vi "RT_lab8.vi"() -> ()   [LabVIEW 2025]
uses:
  states.ctl
panel:
  out "Elements Remaining":u32
  out "Waveform Graph":i16[][](graph)
  out "error out":errorcluster
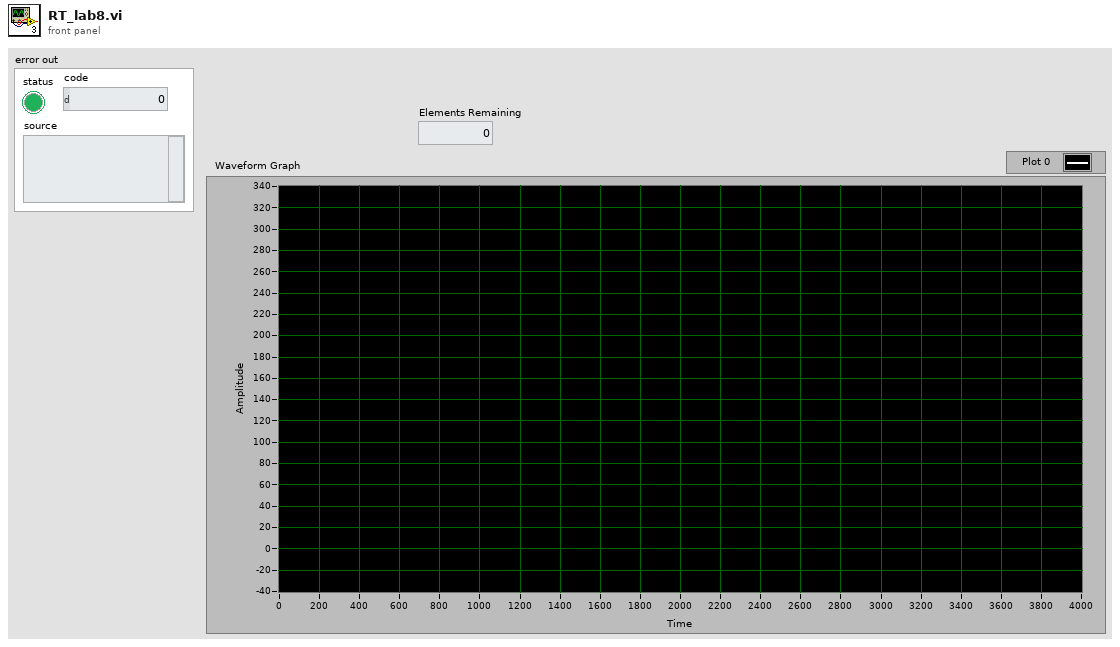
[diagram p1: front panel]
types:
  T1 = typedef "states.ctl" = enum16{"Run", "Connect"}
  T2 = typedef "RT_Cmd.ctl" = cluster{"command":T3, "parameters":T4}
  T3 = typedef "Command.ctl" = enum16{"threshold_config", "manual_trigger", "stop"}
  T4 = typedef "thresholds.ctl" = cluster{"Thr_X":i16, "Thr_Y":i16, "Thr_Z":i16}
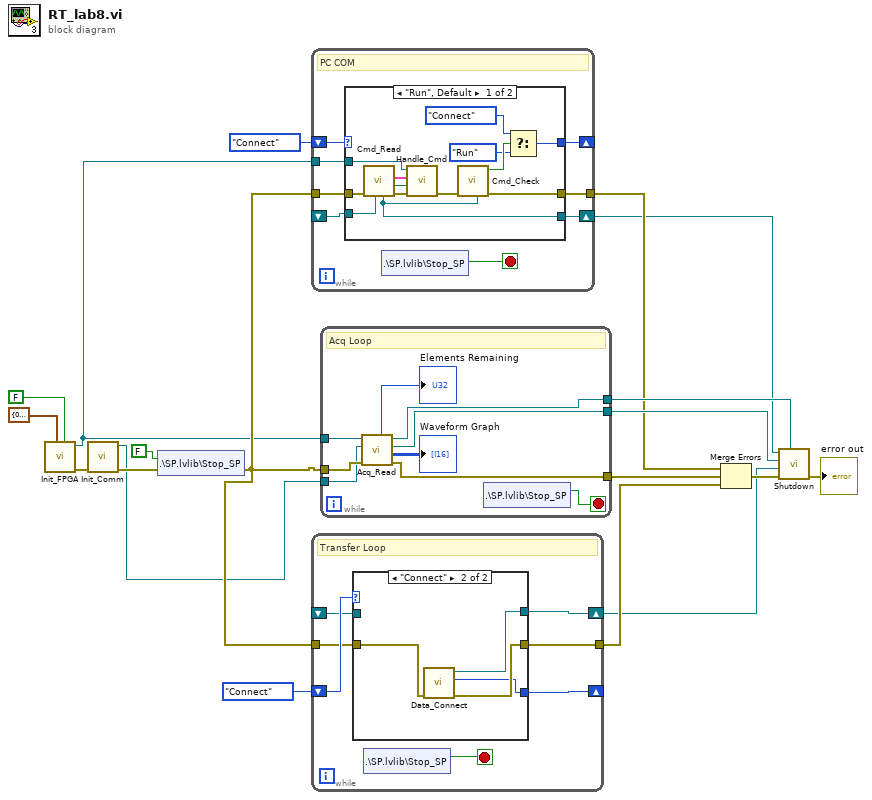
[diagram p0: block diagram]
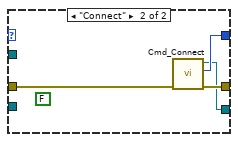
[diagram p2: hidden frame]
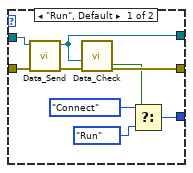
[diagram p3: hidden frame]
diagram:
  n1 = call "Init_FPGA.vi"("manual trigger"=FALSE, "Threshold"=cluster{"Thr_X":i16, "Thr_Y":i16, "Thr_Z":i16} {"Thr_X"=0, "Thr_Y"=0, "Thr_Z"=0}) -> ("error out"=w18:errorcluster, "FPGA VI Reference Out"=w8:refnum<k20>)  [unwired: 8 in]
  n2 = call "Init_Comm.vi"("error in"=w18) -> ("error out"=w14:errorcluster, "rt fifo ref out"=w11:refnum<k33>)  [unwired: 9 in]
  n3 = shared-variable ".\\SP.lvlib\\Stop_SP"(FALSE ("Stop_SP"), error in=w14) -> (error out=w12:errorcluster)
  n4 = while {
    tunnel: w12 -> [w26]
    tunnel: w8 -> [w25]
    shift-right: [w24] -> _
    shift-left: states."Connect" -> [w27]
    tunnel: [w23] -> w3
    shift-right: [w22] -> w1
    shift-left: _ -> [w21]
    stop <- w20 stop-if-true
    # "PC COM"
    n5 = case shown="\"Run\", Default" w27 {
      tunnel: w26 -> [w40 w44]
      tunnel: w25 -> [w38 _]
      tunnel: [w39 w43] -> w23
      tunnel: [w28 w42] -> w24
      tunnel: [w32 w41] -> w22
      tunnel: w21 -> [w33 _]
      frame "Run", Default {
        n6 = call "Cmd_Read.vi"("Refnum in"=w33, "error in (no error)"=w40) -> ("error out"=w35:errorcluster, "timed out?"=w36:bool, "data out"=w37:T2, "Refnum out"=w32:refnum<k21>)  [unwired: 6 in]
        n7 = call "Handle_Cmd.vi"("error in"=w35, "timed out?"=w36, "data IN"=w37, "FPGA VI Reference IN"=w38) -> ("error out"=w34:errorcluster)  [unwired: 6 in, 1 out]
        n8 = call "Cmd_Check.vi"("Refnum in"=w32, "error in (no error)"=w34) -> ("error out"=w39:errorcluster, "disconnected?"=w31:bool)  [unwired: 8 in]
        n9 = Select(t=states."Connect", s=w31, f=states."Run") -> (s? t:f=w28:T1)
      }
      frame "Connect" {
        (unwired) FALSE
        n10 = call "Cmd_Connect.vi"("error in (no error)"=w44) -> ("error out"=w43:errorcluster, "Enum"=w42:T1, "Refnum out"=w41:refnum<k21>)  [unwired: 8 in]
      }
    }
    n11 = shared-variable ".\\SP.lvlib\\Stop_SP"() -> (w20:bool)  [unwired: 1 in, 1 out]
  }
  n12 = while {
    tunnel: w12 -> [w48]
    shift-right: [w47] -> _
    shift-left: states."Connect" -> [w51]
    shift-right: [w50] -> w2
    shift-left: _ -> [w49]
    tunnel: [w46] -> w5
    stop <- w45 stop-if-true
    # "Transfer Loop"
    n13 = case shown="\"Connect\"" w51 {
      tunnel: [w56 w61] -> w50
      tunnel: w49 -> [w59 _]
      tunnel: w48 -> [w60 w63]
      tunnel: [w53 w62] -> w47
      tunnel: [w57 w64] -> w46
      frame "Run", Default {
        n14 = call "Data_Send.vi"("error in (no error)"=w60, "Refnum in"=w59) -> ("error out"=w58:errorcluster, "Refnum out"=w56:refnum<k21>)  [unwired: 8 in]
        n15 = call "Data_Check.vi"("error in (no error)"=w58, "Refnum in"=w56) -> ("error out"=w57:errorcluster, "disconnected?"=w55:bool)  [unwired: 8 in]
        n16 = Select(t=states."Connect", s=w55, f=states."Run") -> (s? t:f=w53:T1)
      }
      frame "Connect" {
        n17 = call "Data_Connect.vi"("error in (no error)"=w63) -> ("error out"=w64:errorcluster, "Enum"=w62:T1, "writer endpoint"=w61:refnum<k21>)  [unwired: 8 in]
      }
    }
    n18 = shared-variable ".\\SP.lvlib\\Stop_SP"() -> (w45:bool)  [unwired: 1 in, 1 out]
  }
  n19 = while {
    tunnel: w8 -> [w73]
    tunnel: w12 -> [w72]
    tunnel: [w71] -> w16
    tunnel: [w69] -> w4
    tunnel: w11 -> [w70]
    tunnel: [w68] -> w15
    stop <- w67 stop-if-true
    # "Acq Loop"
    n20 = call "Acq_Read.vi"("error in (no error)"=w72, "rt fifo ref in"=w70, "Refnum in"=w73) -> ("error out"=w69:errorcluster, "Array"=→"Waveform Graph":i16[][], "rt fifo ref out"=w68:refnum<k33>, "Refnum out"=w71:refnum<k20>, "Elements Remaining"=→"Elements Remaining":u32)  [unwired: 4 in]
    n21 = shared-variable ".\\SP.lvlib\\Stop_SP"() -> (w67:bool)  [unwired: 1 in, 1 out]
  }
  n22 = Merge Errors(w3, w4, w5) -> (w17:errorcluster)
  n23 = call "Shutdown.vi"("Refnum out 3"=w16, "error in (no error)"=w17, 9:"Refnum in"=w2, "rt fifo ref in"=w15, 11:"Refnum in"=w1) -> ("error out"=→"error out":errorcluster)  [unwired: 6 in]
